vi "Viewport.vi"   [LabVIEW 2024]
uses:
  Navigator/Navigator.lvclass
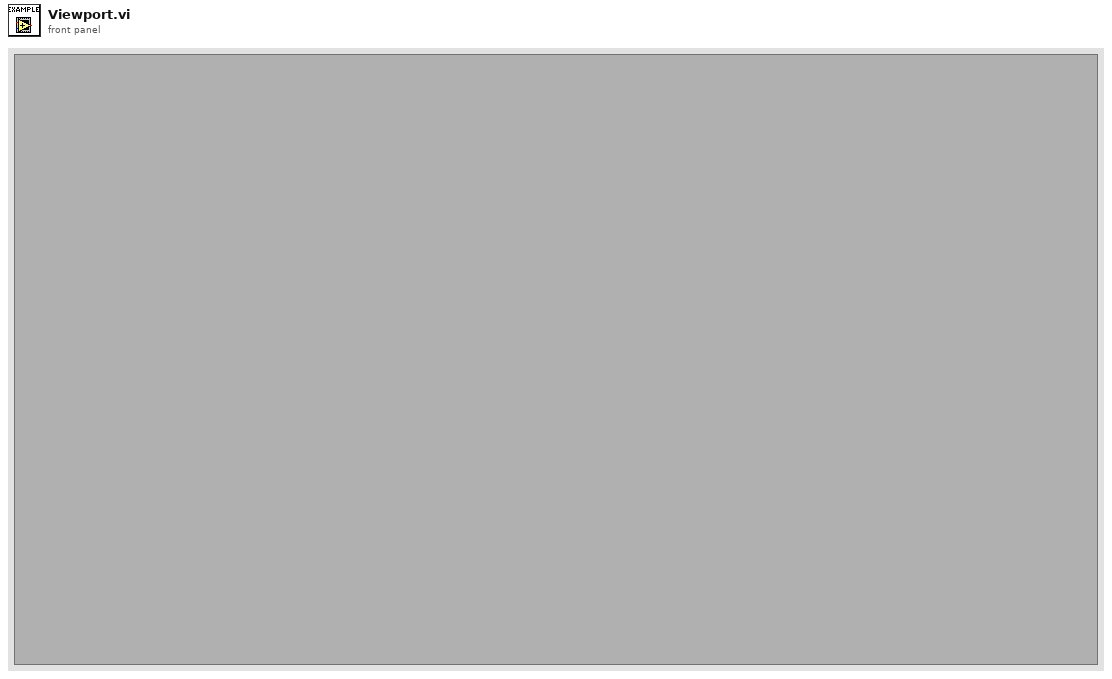
[diagram p1: front panel]
types:
  T1 = typedef "Navigator.lvclass/Route.ctl" = cluster{"Name":string, "Path":path, "Builder":refnum<class "NavigatableView.lvclass">}
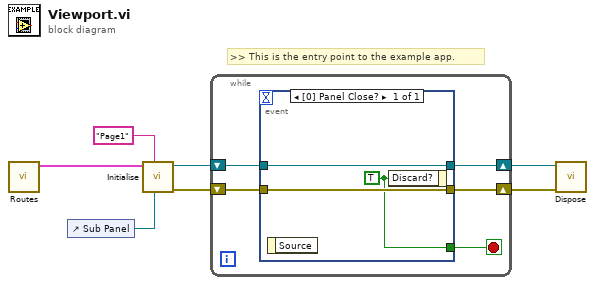
[diagram p0: block diagram]
diagram:
  # ">> This is the entry point to the example app."
  n1 = call "Routes.vi"() -> ("Routes"=w2:T1[])  [unwired: 11 in]
  n2 = control-ref of="Sub Panel"() -> (w7:refnum<vi>)
  n3 = call "Initialise.vi"("SubPanelReference"=w7, "InitialRoute"="Page1", "Routes"=w2) -> ("error out"=w5:errorcluster, "Navigator out"=w6:refnum<class "Navigator.lvclass">)  [unwired: 7 in]
  n4 = while {
    shift-right: [w10] -> w4
    shift-left: w6 -> [w12]
    shift-right: [w9] -> w3
    shift-left: w5 -> [w11]
    stop <- w8 stop-if-true
    n5 = event shown="[0] Panel Close?" {
      selector: _ -> [_]
      dyn-events: _ -> [_]
      timeout: _ -> [_]
      tunnel: w12 -> [w15]
      tunnel: w11 -> [w14]
      tunnel: [w15] -> w10
      tunnel: [w14] -> w9
      tunnel: [w13] -> w8
      event Panel Close? {
        w13 = TRUE ("Discard?")
        n6 = event-data() -> ()  [unwired: 1 in, 1 out]
        n7 = event-data("Discard?"=w13) -> ()  [unwired: 1 in, 1 out]
      }
    }
  }
  n8 = call "Dispose.vi"("error in (no error)"=w3, "Navigator in"=w4) -> ()  [unwired: 8 in, 2 out]
